vi "lvmcp_libsave.vi"(11 "library":path) -> (0 "error out":errorcluster)   [LabVIEW 2015]
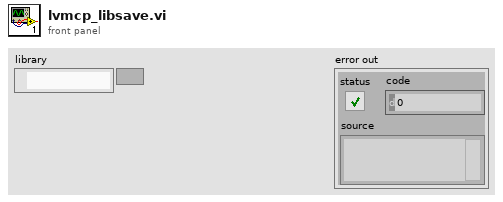
[diagram p1: front panel]
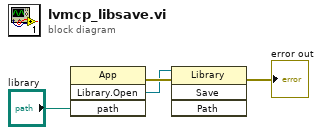
[diagram p0: block diagram]
diagram:
  n1 = invoke class="App" method="Library.Open"("path"="library") -> (error out=w3:errorcluster, "Open Library"=w1:refnum<vi>)  [unwired: 3 in, 2 out]
  n2 = invoke class="Library" method="Save"(reference=w1, error in=w3) -> (error out=→"error out":errorcluster)  [unwired: 2 in, 3 out]
